vi "FRC_read utility xml files.vi"() -> (8 "utilities data array":T1[](array[typedef]))   [LabVIEW 2023, in "GettingStartedWindow.lvlib"]
uses:
  <resource>/modes/FRC/GSW/GettingStartedWindow.lvlib
  <resource>/modes/FRC/GSW/FRC_UtilitiesData.ctl
  <vilib>/Utility/sysdir.llb/System Directory Type.ctl
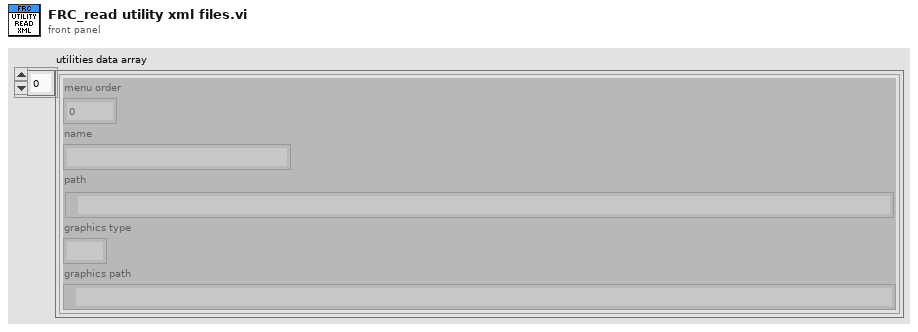
[diagram p1: front panel]
types:
  T1 = typedef "GettingStartedWindow.lvlib/FRC_UtilitiesData.ctl" = cluster{"menu order":i32, "name":string, "path":path, "graphics type":string, "graphics path":path}
  T2 = typedef "System Directory Type.ctl" = i32
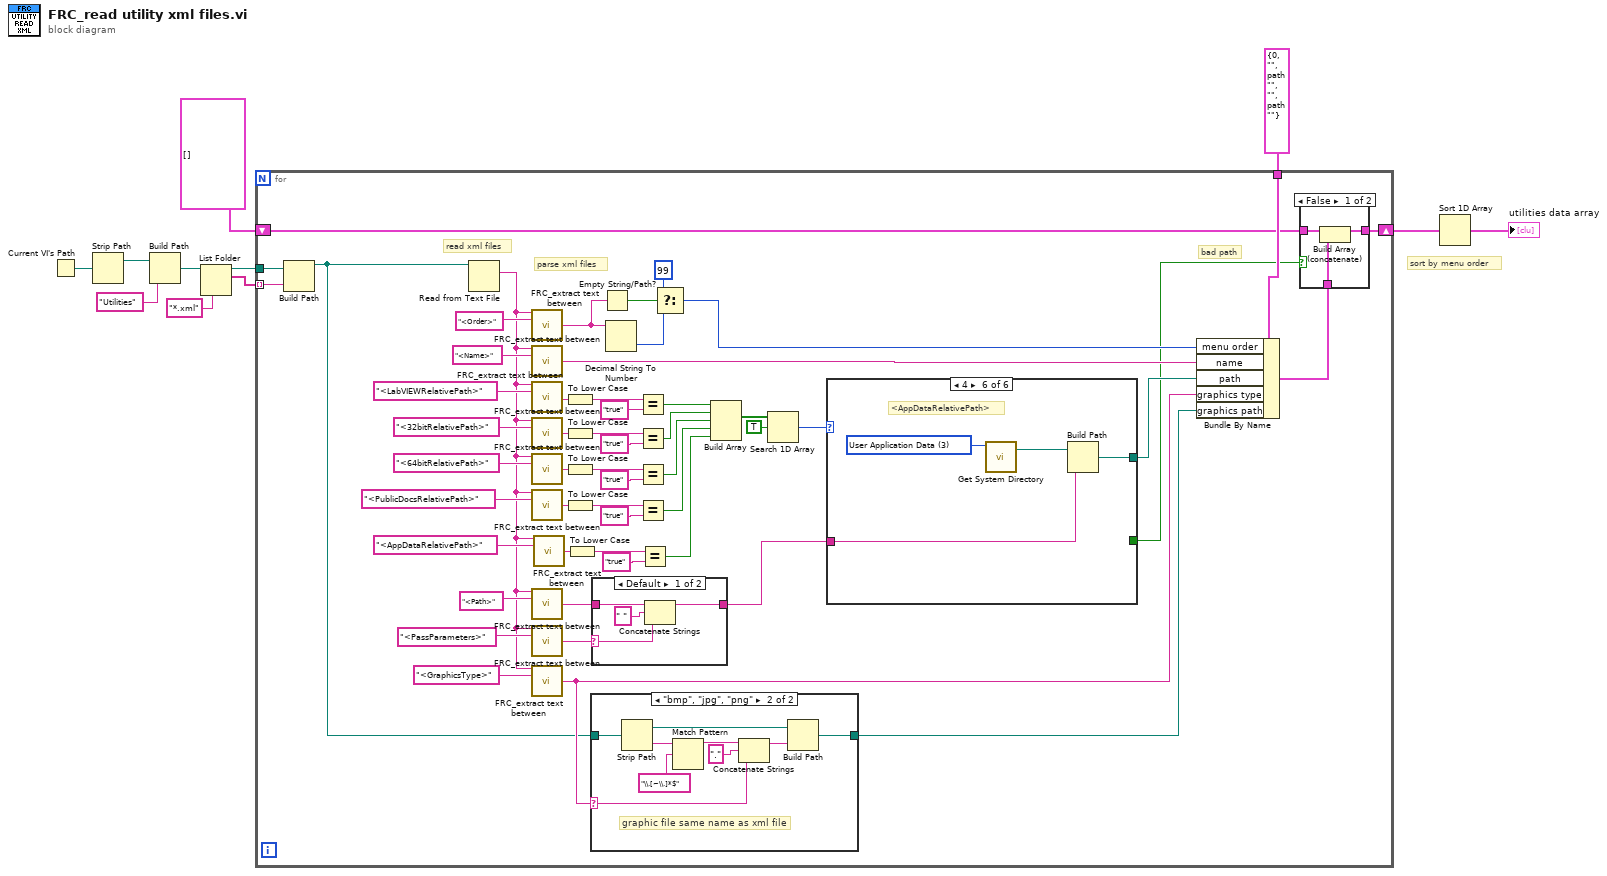
[diagram p0: block diagram]
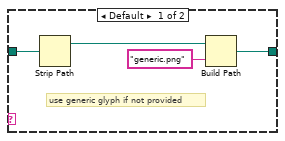
[diagram p3: hidden frame]
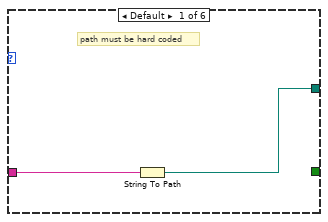
[diagram p5: hidden frame]
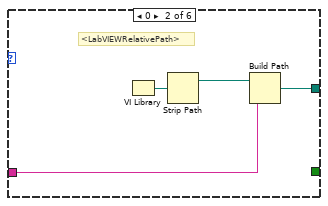
[diagram p6: hidden frame]
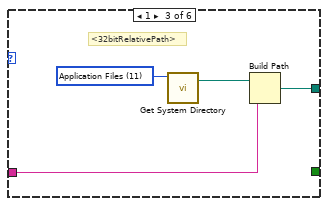
[diagram p7: hidden frame]
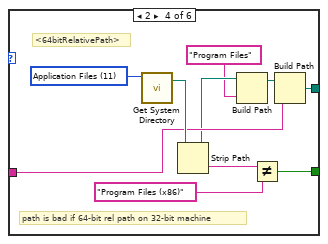
[diagram p8: hidden frame]
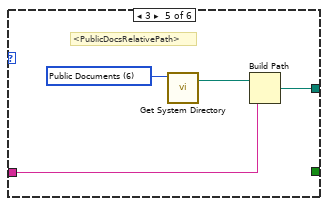
[diagram p9: hidden frame]
diagram:
  # "sort by menu order"
  n1 = Current VI's Path() -> (path=w1:path)
  n2 = Strip Path(path=w1) -> (stripped path=w11:path)  [unwired: 1 out]
  n3 = Build Path(base path=w11, name or relative path="Utilities") -> (appended path=w4:path)
  n4 = List Folder(path=w4, pattern="*.xml") -> (path out=w8:path, filenames=w7:string[])  [unwired: 2 in, 2 out]
  n5 = for {
    tunnel: w8 -> [w65]
    tunnel: w7 -> [w64] mode=indexing
    tunnel: T1 {"menu order"=0, "name"="", "path"=path "", "graphics type"="", "graphics path"=path ""} ("utilities data") -> [w62]
    shift-right: [w19] -> w5
    shift-left: T1[] [] -> [w21]
    # "bad path"
    # "read xml files"
    # "parse xml files"
    n6 = Build Path(base path=w65, name or relative path=w64) -> (appended path=w30:path)
    n7 = Read from Text File(file (use dialog)=w30) -> (text=w13:string)  [unwired: 3 in, 3 out]
    n8 = call <resource>:"FRC_extract text between.vi"("string"=w13, "after this text"="<Order>") -> ("extracted text"=w27:string)  [unwired: 10 in, 3 out]
    n9 = call <resource>:"FRC_extract text between.vi"("string"=w13, "after this text"="<Name>") -> ("extracted text"=w61:string)  [unwired: 10 in, 3 out]
    n10 = call <resource>:"FRC_extract text between.vi"("string"=w13, "after this text"="<LabVIEWRelativePath>") -> ("extracted text"=w51:string)  [unwired: 10 in, 3 out]
    n11 = call <resource>:"FRC_extract text between.vi"("string"=w13, "after this text"="<32bitRelativePath>") -> ("extracted text"=w57:string)  [unwired: 10 in, 3 out]
    n12 = call <resource>:"FRC_extract text between.vi"("string"=w13, "after this text"="<64bitRelativePath>") -> ("extracted text"=w48:string)  [unwired: 10 in, 3 out]
    n13 = call <resource>:"FRC_extract text between.vi"("string"=w13, "after this text"="<PublicDocsRelativePath>") -> ("extracted text"=w45:string)  [unwired: 10 in, 3 out]
    n14 = call <resource>:"FRC_extract text between.vi"("string"=w13, "after this text"="<Path>") -> ("extracted text"=w32:string)  [unwired: 10 in, 3 out]
    n15 = call <resource>:"FRC_extract text between.vi"("string"=w13, "after this text"="<PassParameters>") -> ("extracted text"=w33:string)  [unwired: 10 in, 3 out]
    n16 = call <resource>:"FRC_extract text between.vi"("string"=w13, "after this text"="<GraphicsType>") -> ("extracted text"=w31:string)  [unwired: 10 in, 3 out]
    n17 = call <resource>:"FRC_extract text between.vi"("string"=w13, "after this text"="<AppDataRelativePath>") -> ("extracted text"=w15:string)  [unwired: 10 in, 3 out]
    n18 = To Lower Case(string=w51) -> (all lower case string=w52:string)
    n19 = To Lower Case(string=w57) -> (all lower case string=w56:string)
    n20 = To Lower Case(string=w48) -> (all lower case string=w49:string)
    n21 = To Lower Case(string=w45) -> (all lower case string=w44:string)
    n22 = To Lower Case(string=w15) -> (all lower case string=w16:string)
    n23 = case shown="\"bmp\", \"jpg\", \"png\"" w31 {
      selector: w31 -> [_ w76]
      tunnel: w30 -> [w73 w81]
      tunnel: [w72 w74] -> w29
      frame Default {
        # "use generic glyph if not provided"
        n24 = Strip Path(path=w73) -> (stripped path=w71:path)  [unwired: 1 out]
        n25 = Build Path(base path=w71, name or relative path="generic.png") -> (appended path=w72:path)
      }
      frame "bmp", "jpg", "png" {
        # "graphic file same name as xml file"
        n26 = Strip Path(path=w81) -> (stripped path=w82:path, name=w79:string)
        n27 = Match Pattern(string=w79, regular expression="\\.[~\\.]*$") -> (before substring=w78:string)  [unwired: 4 out]
        n28 = Concatenate Strings(w78, "." ("string"), w76) -> (w75:string)
        n29 = Build Path(base path=w82, name or relative path=w75) -> (appended path=w74:path)
      }
    }
    n30 = case shown="Default" w33 {
      selector: w33 -> [w83 _]
      tunnel: w32 -> [w86 w87]
      tunnel: [w85 w87] -> w18
      frame Default {
        n31 = Concatenate Strings(w86, " " ("string"), w83) -> (w85:string)
      }
      frame "" {
      }
    }
    n32 = Empty String/Path?(string/path=w27) -> (empty?=w26:bool)
    n33 = Decimal String To Number(string=w27) -> (number=w24:i32)  [unwired: 2 in, 1 out]
    n34 = Equal?(x=w52, y="true") -> (x = y?=w41:bool)
    n35 = Equal?(x=w56, y="true") -> (x = y?=w40:bool)
    n36 = Equal?(x=w49, y="true") -> (x = y?=w39:bool)
    n37 = Equal?(x=w44, y="true") -> (x = y?=w38:bool)
    n38 = Equal?(x=w16, y="true") -> (x = y?=w12:bool)
    n39 = Select(t=99, s=w26, f=w24) -> (s? t:f=w23:i32)
    n40 = Build Array(w41, w40, w39, w38, w12) -> (w37:bool[])
    n41 = Search 1D Array(1D array=w37, element=TRUE) -> (index of element=w35:i32)  [unwired: 1 in]
    n42 = case shown="4" w35 {
      tunnel: w18 -> [w89 w91 w97 w101 w111 w115]
      tunnel: [w88 w90 w96 w107 w110 w114] -> w34
      tunnel: [_ _ _ w102 _ _] -> w22
      frame Default {
        # "path must be hard coded"
        n43 = String To Path(string=w89) -> (path=w88:path)
      }
      frame 0 {
        # "<LabVIEWRelativePath>"
        n44 = VI Library() -> (path=w93:path)
        n45 = Strip Path(path=w93) -> (stripped path=w92:path)  [unwired: 1 out]
        n46 = Build Path(base path=w92, name or relative path=w91) -> (appended path=w90:path)
      }
      frame 1 {
        w95 = T2 11 items=["User Home"=0, "User Desktop"=1, "User Documents"=2, "User Application Data"=3, "User Preferences"=4, "User Temporary"=5, "Public Documents"=6, "Public Application Data"=7, "Public Preferences"=8, "Public Cache"=13, "System Core Libraries"=9, "System Installed Libraries"=10, "Application Files"=11, "Boot Volume Root"=12] ("system directory type")
        # "<32bitRelativePath>"
        n47 = call <vilib>:"Get System Directory.vi"("system directory type"=w95) -> ("system directory"=w94:path)  [unwired: 10 in]
        n48 = Build Path(base path=w94, name or relative path=w97) -> (appended path=w96:path)
      }
      frame 2 {
        w106 = T2 11 items=["User Home"=0, "User Desktop"=1, "User Documents"=2, "User Application Data"=3, "User Preferences"=4, "User Temporary"=5, "Public Documents"=6, "Public Application Data"=7, "Public Preferences"=8, "Public Cache"=13, "System Core Libraries"=9, "System Installed Libraries"=10, "Application Files"=11, "Boot Volume Root"=12] ("system directory type")
        # "path is bad if 64-bit rel path on 32-bit machine"
        # "<64bitRelativePath>"
        n49 = call <vilib>:"Get System Directory.vi"("system directory type"=w106) -> ("system directory"=w105:path)  [unwired: 10 in]
        n50 = Strip Path(path=w105) -> (stripped path=w99:path, name=w104:string)
        n51 = Build Path(base path=w99, name or relative path="Program Files" ("y")) -> (appended path=w100:path)
        n52 = Not Equal?(x=w104, y="Program Files (x86)") -> (x != y?=w102:bool)
        n53 = Build Path(base path=w100, name or relative path=w101) -> (appended path=w107:path)
      }
      frame 3 {
        w109 = T2 6 items=["User Home"=0, "User Desktop"=1, "User Documents"=2, "User Application Data"=3, "User Preferences"=4, "User Temporary"=5, "Public Documents"=6, "Public Application Data"=7, "Public Preferences"=8, "Public Cache"=13, "System Core Libraries"=9, "System Installed Libraries"=10, "Application Files"=11, "Boot Volume Root"=12] ("system directory type")
        # "<PublicDocsRelativePath>"
        n54 = call <vilib>:"Get System Directory.vi"("system directory type"=w109) -> ("system directory"=w108:path)  [unwired: 10 in]
        n55 = Build Path(base path=w108, name or relative path=w111) -> (appended path=w110:path)
      }
      frame 4 {
        w113 = T2 3 items=["User Home"=0, "User Desktop"=1, "User Documents"=2, "User Application Data"=3, "User Preferences"=4, "User Temporary"=5, "Public Documents"=6, "Public Application Data"=7, "Public Preferences"=8, "Public Cache"=13, "System Core Libraries"=9, "System Installed Libraries"=10, "Application Files"=11, "Boot Volume Root"=12] ("system directory type")
        # "<AppDataRelativePath>"
        n56 = call <vilib>:"Get System Directory.vi"("system directory type"=w113) -> ("system directory"=w112:path)  [unwired: 10 in]
        n57 = Build Path(base path=w112, name or relative path=w115) -> (appended path=w114:path)
      }
    }
    n58 = Bundle By Name(cluster=w62, "menu order"=w23, "name"=w61, "path"=w34, "graphics type"=w31, "graphics path"=w29) -> (w20:T1)
    n59 = case shown="False" w22 {
      tunnel: w21 -> [w68 w69]
      tunnel: w20 -> [w67 _]
      tunnel: [w66 w69] -> w19
      frame False {
        n60 = Build Array (concatenate)(w68, w67) -> (w66:T1[])
      }
      frame True {
      }
    }
  }
  n61 = Sort 1D Array(array=w5) -> (sorted array=→"utilities data array":T1[])
